vi "Cleanup.vi"(8 "error in (no error)":errorcluster, 11 "CIFPlugin in":refnum<class "CAN_Writer_CANsub_Plugin.lvclass">) -> (0 "error out":errorcluster, 3 "CIFPlugin out":refnum<class "CAN_Writer_CANsub_Plugin.lvclass">)   [LabVIEW 2021, in "CAN_Writer_CANsub_Plugin.lvclass"]
uses:
  CAN_Writer_CANsub_Plugin.lvclass
  CAN_Writer_CANsub_Plugin.lvclass/CAN_Writer_CANsub_Plugin.ctl
  <vilib>/CIF Foundation/CIF XNET CAN RW/XNET CAN RW.lvclass
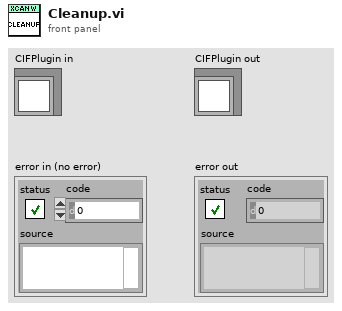
[diagram p1: front panel]
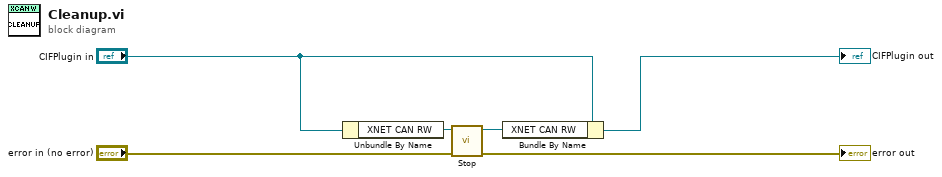
[diagram p0: block diagram]
diagram:
  n1 = Unbundle By Name("CIFPlugin in") -> ("XNET CAN RW"=w6:refnum<class "XNET CAN RW.lvclass">)
  n2 = call-dynamic "Stop.vi"("error in (no error)"="error in (no error)", "XNET_CAN_RW in"=w6) -> ("error out"=→"error out":errorcluster, "XNET_CAN_RW out"=w5:refnum<class "XNET CAN RW.lvclass">)  [unwired: 8 in]
  n3 = Bundle By Name(cluster="CIFPlugin in", "XNET CAN RW"=w5) -> (→"CIFPlugin out":refnum<class "CAN_Writer_CANsub_Plugin.lvclass">)
